vi "ActionVIOnLoad.vi"(8 "error in (no error)":errorcluster, 11 "Device Item Ref in":T1 format="%.0x") -> (0 "error out":errorcluster, 3 "Device Item Ref out":T1 format="%.0x")   [LabVIEW 2020, in "FPGA Addon System Explorer.lvlib"]
uses:
  FPGA Addon System Explorer.lvlib
  <vilib>/NI VeriStand/Custom Device API/Custom Device Item Ref.ctl
  Addon Shared/Types/FG Action.ctl
  Addon Shared/SubVIs/Constants.vi
  <vilib>/NI VeriStand/Custom Device API/Get Item Property (Path).vi
  <vilib>/NI VeriStand/Custom Device API/Get Item Property (String).vi
  <vilib>/NI VeriStand/Custom Device API/Get Item Property (Boolean).vi
  <vilib>/NI VeriStand/Custom Device API/NI VeriStand - Set Item Property.vi
  <vilib>/NI VeriStand/Custom Device API/Set Item Property (Path).vi
  <vilib>/NI VeriStand/Custom Device API/Set Item Property (String).vi
  <vilib>/NI VeriStand/Custom Device API/Set Item Property (Boolean).vi
  <vilib>/NI VeriStand/Custom Device API/Get Item Property (Dependent File).vi
  Addon Shared/FPGA Addon Shared.lvlib
  <vilib>/NI VeriStand/Custom Device API/Custom Device API.lvlib
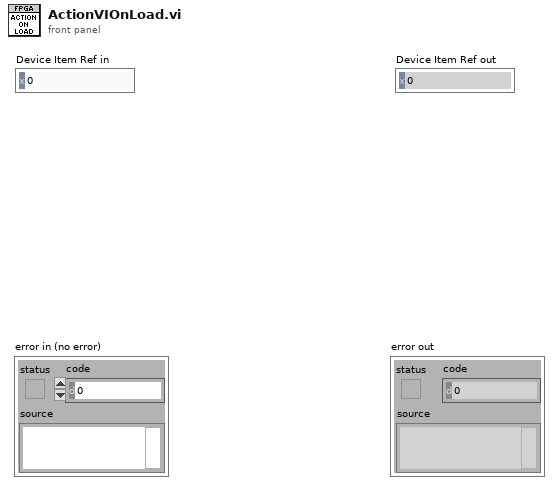
[diagram p1: front panel]
types:
  T1 = typedef "Custom Device API.lvlib/Custom Device Item Ref.ctl" = u64
  T2 = typedef "FPGA Addon Shared.lvlib/FG Action.ctl" = enum8{"GET", "SET"}
  T3 = typedef "FPGA Addon Shared.lvlib/FPGA Settings.ctl" = cluster{"Bitfile path":path, "RIO Device Address":string, "Group":bool}
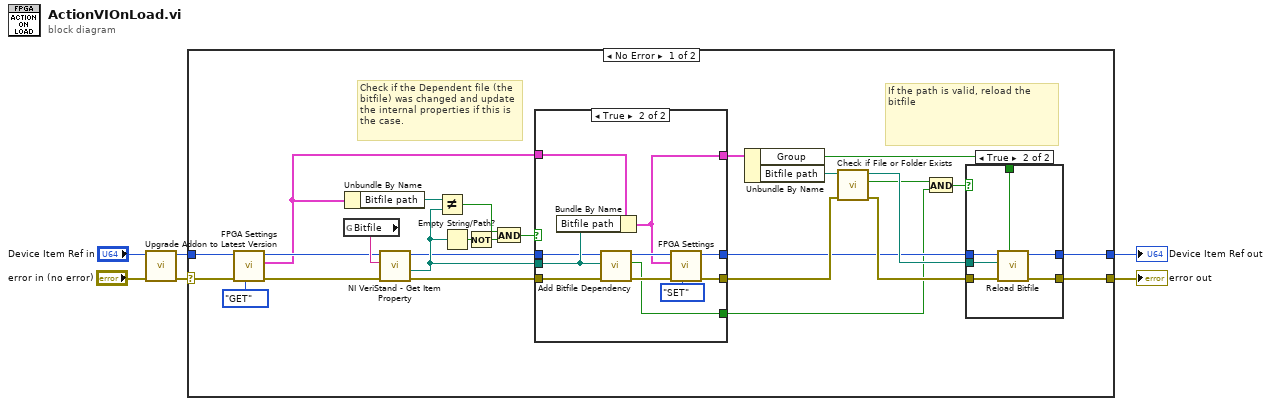
[diagram p0: block diagram]
diagram:
  n1 = call "Upgrade Addon to Latest Version.vi"("error in (no error)"="error in (no error)", "Device Item Ref in in"="Device Item Ref in") -> ("error out"=w1:errorcluster, "Device Item Ref out"=w4:T1)  [unwired: 8 in]
  n2 = case shown="No Error" w1 {
    selector: w1 -> [w32 w56]
    tunnel: w4 -> [w33 w57]
    tunnel: [w19 w57] -> w3
    tunnel: [w18 w56] -> w2
    frame No Error {
      # "If the path is valid, reload the bitfile"
      # "Check if the Dependent file (the bitfile) was changed and update the internal properties if this is the case."
      n3 = call "FPGA Settings.vi"("Action"=FG_Action."GET", "error in (no error)"=w32, "Item Ref"=w33) -> ("error out"=w22:errorcluster, "FPGA Settings"=w20:T3, "Item Ref out"=w21:T1)  [unwired: 6 in]
      n4 = global read "Constants.vi" "Bitfile"() -> (w23:string)
      n5 = Unbundle By Name(w20) -> ("Bitfile path"=w27:path)
      n6 = call-poly <vilib>:"NI VeriStand - Get Item Property.vi"("error in (no error)"=w22, "Property Name"=w23, "Item Ref in"=w21) -> ("error out"=w24:errorcluster, "Path"=w28:path, "Item Ref out"=w25:T1)  [unwired: 4 in, 2 out]
      n7 = Not Equal?(x=w27, y=w28) -> (x != y?=w30:bool)
      n8 = Empty String/Path?(string/path=w28) -> (empty?=w26:bool)
      n9 = Not(x=w26) -> (.not. x?=w29:bool)
      n10 = And(x=w30, y=w29) -> (x .and. y?=w10:bool)
      n11 = case shown="True" w10 {
        tunnel: w28 -> [_ w47]
        tunnel: w25 -> [w35 w46]
        tunnel: w24 -> [w34 w45]
        tunnel: w20 -> [w36 w44]
        tunnel: [w34 w40] -> w14
        tunnel: [w35 w39] -> w13
        tunnel: [w36 w38] -> w12
        tunnel: [_ w37] -> w7
        frame False {
        }
        frame True {
          n12 = Bundle By Name(cluster=w44, "Bitfile path"=w47) -> (w38:T3)
          n13 = call "Add Bitfile Dependency.vi"("error in (no error)"=w45, "Path"=w47, "Item Ref in"=w46) -> ("error out"=w41:errorcluster, "bitfile changed"=w37:bool, "Item Ref out"=w42:T1)  [unwired: 6 in]
          n14 = call "FPGA Settings.vi"("Action"=FG_Action."SET", "error in (no error)"=w41, "FPGA Settings"=w38, "Item Ref"=w42) -> ("error out"=w40:errorcluster, "Item Ref out"=w39:T1)  [unwired: 5 in, 1 out]
        }
      }
      n15 = Unbundle By Name(w12) -> ("Group"=w11:bool, "Bitfile path"=w15:path)
      n16 = call <vilib>:"Check if File or Folder Exists.vi"("error in (no error)"=w14, "path"=w15) -> ("error out"=w17:errorcluster, "file or folder exists?"=w9:bool, "dup path"=w16:path)  [unwired: 7 in]
      n17 = And(x=w9, y=w7) -> (x .and. y?=w8:bool)
      n18 = case shown="True" w8 {
        tunnel: w17 -> [w48 w55]
        tunnel: w16 -> [_ w54]
        tunnel: w13 -> [w49 w53]
        tunnel: [w48 w52] -> w18
        tunnel: [w49 w51] -> w19
        tunnel: w11 -> [_ w50]
        frame False {
        }
        frame True {
          n19 = call "Reload Bitfile.vi"("Group"=w50, "error in (no error)"=w55, "NewVal"=w54, "Item Ref in"=w53) -> ("error out"=w52:errorcluster, "Section Ref out"=w51:T1)  [unwired: 6 in]
        }
      }
    }
    frame Error {
    }
  }
  "error out" <- w2
  "Device Item Ref out" <- w3
